vi "testBatchDetection.vi"() -> ()   [LabVIEW 2025]
uses:
  tcv/def/devices.ctl
  dl/initModelv2Params.ctl
  dl/dl.lvclass
  tcv/tcv.lvclass
panel:
  out "seg":T1(plugin-control)
  out "SetDevice":string
  out "runSucc":i32
  out "loadImgSucc":string
  out "maskCounts":i32[](array[numeric])
  out "bbCounts":i32[](array[numeric])
  in  "initModelv2Params":T2={"modelH"=736, "modelW"=1280, "frameH"=1080, "frameW"=1920, "batchSize"=1, "conf"=0.6, "iou"=0.55}
  in  "modelpath":path=path "D:/Test/adslvPackageDev/models/nws_736_1280_b1_gpu.torchscript"
  out "Image":T1(plugin-control)
  in  "path":path=path "D:/Test/adslvPackageDev/images/wsn"
  in  "devices":T3=enum."GPU0"
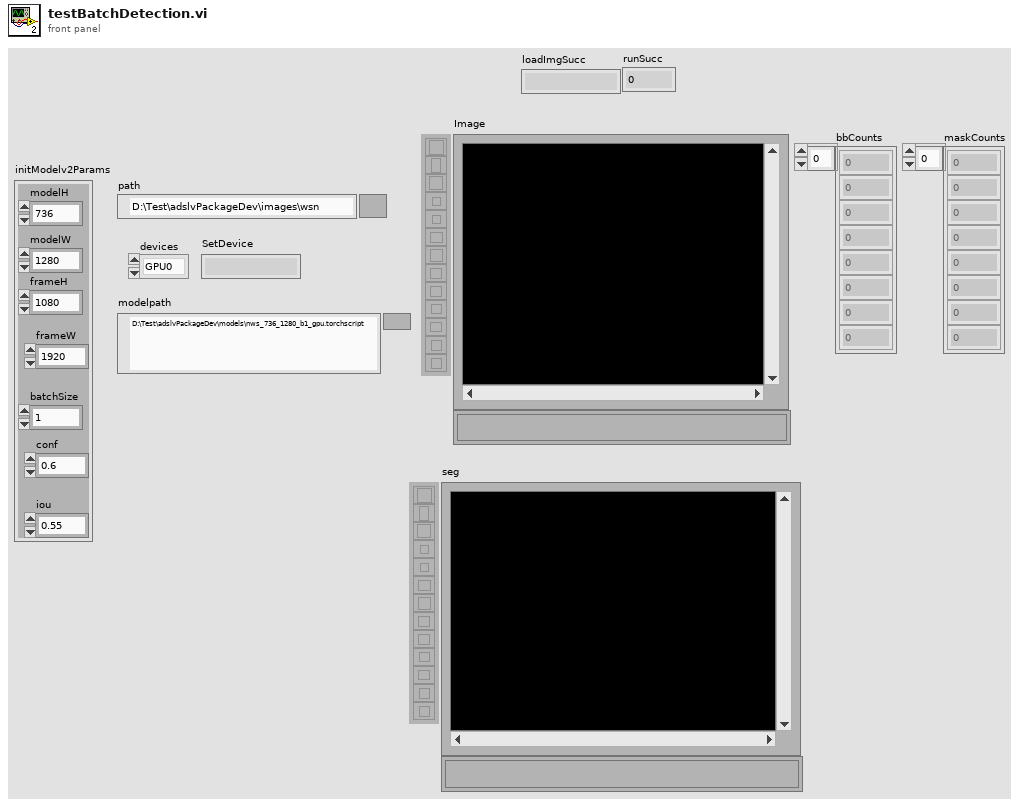
[diagram p1: front panel]
types:
  T1 = typedef "IMAQ Image.ctl" = refnum<image>
  T2 = typedef "dl.lvlib/dl.lvclass/initModelv2Params.ctl" = cluster{"modelH":i32, "modelW":i32, "frameH":i32, "frameW":i32, "batchSize":i32, "conf":sgl, "iou":sgl}
  T3 = typedef "tcv.lvlib/tcv.lvclass/devices.ctl" = enum16{"CPU", "GPU0"}
  T4 = typedef "dl.lvlib/dl.lvclass/ImageDetections.ctl" = cluster{"Detections":T5[]}
  T5 = typedef "dl.lvlib/dl.lvclass/detect.ctl" = cluster{"x1":sgl, "y1":sgl, "x2":sgl, "y2":sgl, "cnf":sgl, "clsID":i32}
  T6 = typedef "dl.lvlib/dl.lvclass/ImageMasks.ctl" = cluster{"Polygons ":T7[]}
  T7 = typedef "dl.lvlib/dl.lvclass/Polygon.ctl" = cluster{"Vertices":T8[]}
  T8 = typedef "dl.lvlib/dl.lvclass/LVPointInt.ctl" = cluster{"x":i32, "y":i32}
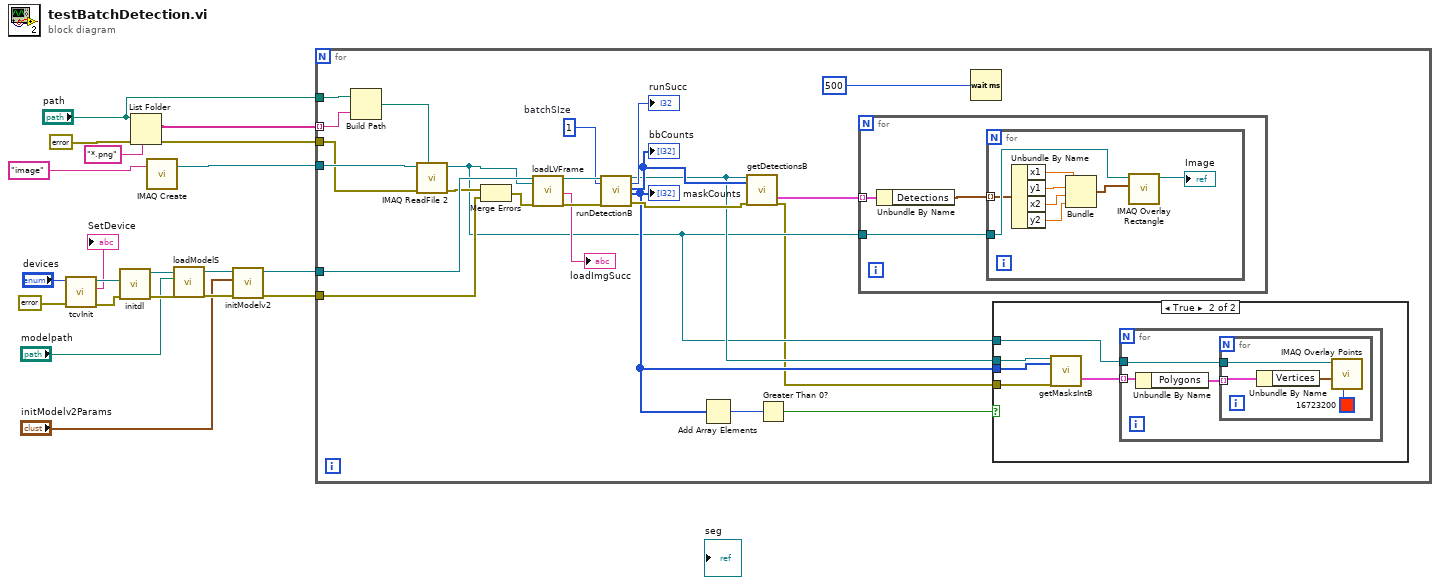
[diagram p0: block diagram]
diagram:
  n1 = call "tcvInit.vi"("error in"=errorcluster {"status"=FALSE, "code"=0, "source"=""}, "devices"="devices") -> ("error out"=w10:errorcluster, "SetDevice"=→"SetDevice":string, "tcv out"=w11:refnum<class "tcv.lvclass">)  [unwired: 7 in]
  n2 = call "initdl.vi"("error in (no error)"=w10, "tcv in"=w11) -> ("error out"=w8:errorcluster, "dl out"=w9:refnum<class "dl.lvclass">)  [unwired: 8 in]
  n3 = List Folder(path="path", pattern="*.png", error in=errorcluster {"status"=FALSE, "code"=0, "source"=""}) -> (filenames=w16:string[], error out=w12:errorcluster)  [unwired: 1 in, 2 out]
  n4 = call "IMAQ Create"("Image Name"="image") -> ("New Image"=w13:T1)  [unwired: 4 in, 1 out]
  n5 = call-dynamic "loadModelS.vi"("error in (no error)"=w8, "modelpath"="modelpath", "dl in"=w9) -> ("error out"=w5:errorcluster, "dl out"=w6:refnum<class "dl.lvclass">)  [unwired: 6 in, 1 out]
  n6 = call-dynamic "initModelv2.vi"("error in (no error)"=w5, "initModelv2Params"="initModelv2Params", "dl in"=w6) -> ("error out"=w2:errorcluster, "dl out"=w3:refnum<class "dl.lvclass">)  [unwired: 7 in]
  n7 = for {
    tunnel: "path" -> [w44]
    tunnel: w16 -> [w43] mode=indexing
    tunnel: w13 -> [w41]
    tunnel: w12 -> [w39]
    tunnel: w3 -> [w38]
    tunnel: w2 -> [w36]
    w32 = 1  # batchSIze
    n8 = Build Path(base path=w44, name or relative path=w43) -> (appended path=w40:path)
    n9 = call "IMAQ ReadFile 2"("File Path"=w40, "error in (no error)"=w39, "Image"=w41) -> ("error out"=w37:errorcluster, "Image Out"=w23:T1)  [unwired: 4 in, 3 out]
    n10 = Merge Errors(w37, w36) -> (w35:errorcluster)
    n11 = call-dynamic "loadLVFrame.vi"("tcv in"=w38, "Image"=w23, "error in (no error)"=w35) -> ("tcv out"=w34:refnum<class "dl.lvclass">, "loadImgSucc"=→"loadImgSucc":string, "error out"=w33:errorcluster)  [unwired: 13 in, 1 out]
    n12 = call-dynamic "runDetectionB.vi"("dl in"=w34, "batchSIze"=w32, "error in (no error)"=w33) -> ("dl out"=w27:refnum<class "dl.lvclass">, "runSucc"=→"runSucc":i32, "bbCounts"=w29:i32[], "maskCounts"=w25:i32[], "error out"=w28:errorcluster)  [unwired: 12 in]
    "bbCounts" <- w29
    "maskCounts" <- w25
    n13 = Add Array Elements(numeric array=w25) -> (sum=w24:i32)
    n14 = call-dynamic "getDetectionsB.vi"("dl in"=w27, "bbCounts"=w29, "error in (no error)"=w28) -> ("BatchDetections"=w22:T4[], "error out"=w21:errorcluster)  [unwired: 11 in, 4 out]
    n15 = Greater Than 0?(x=w24) -> (x > 0?=w26:bool)
    n16 = for {
      tunnel: w23 -> [w47]
      tunnel: w22 -> [w46] mode=indexing
      n17 = Unbundle By Name(w46) -> ("Detections"=w45:T5[])
      n18 = for {
        tunnel: w47 -> [w50]
        tunnel: w45 -> [w48] mode=indexing
        n19 = Unbundle By Name(w48) -> ("x1"=w55:sgl, "y1"=w54:sgl, "x2"=w53:sgl, "y2"=w52:sgl)
        n20 = Bundle("x1"=w55, "y1"=w54, "x2"=w53, "y2"=w52) -> (w51:cluster{"x1":sgl, "y1":sgl, "x2":sgl, "y2":sgl})  [unwired: 1 in]
        n21 = call "IMAQ Overlay Rectangle"("Rectangle"=w51, "Image"=w50) -> ("Image Out"=→"Image":T1)  [unwired: 8 in, 1 out]
      }
    }
    n22 = Wait (ms)(milliseconds to wait=u32 500) -> ()  [unwired: 1 out]
    n23 = case shown="True" w26 {
      tunnel: w27 -> [_ w60]
      tunnel: w25 -> [_ w59]
      tunnel: w23 -> [_ w57]
      tunnel: w21 -> [_ w56]
      frame False {
      }
      frame True {
        n24 = call-dynamic "getMasksIntB.vi"("dl in"=w60, "maskCounts"=w59, "error in (no error)"=w56) -> ("BatchMasks"=w58:T6[])  [unwired: 11 in, 5 out]
        n25 = for {
          tunnel: w58 -> [w63] mode=indexing
          tunnel: w57 -> [w62]
          n26 = Unbundle By Name(w63) -> ("Polygons"=w61:T7[])
          n27 = for {
            tunnel: w62 -> [w67]
            tunnel: w61 -> [w65] mode=indexing
            n28 = Unbundle By Name(w65) -> ("Vertices"=w64:T8[])
            n29 = call "IMAQ Overlay Points"("Color"=u32 16723200, "Array of Points"=w64, "Image"=w67) -> ()  [unwired: 7 in, 2 out]
          }
        }
      }
    }
  }
